vi "GDSLvIcon_AnalyseViIcon.vi"(1 "ViRef/LvCLassRef/LvLibRef/ViPath/2D_Image":variant, 3 "DoATextOCR(False)":bool, 5 "error in (no error)":errorcluster) -> (6 "BodyTextColor":u32(colorbox), 7 "Splitter0px":bool, 8 "HeaderTextColor":u32(colorbox), 9 "BodyText(OCR)":string, 10 "FrameColor":u32(colorbox), 11 "HeadText(OCR)":string, 12 "FrameThickness(1)":u32=1, 13 "ValidHeaderIcon":bool, 14 "DefaultIcon":bool, 15 "HeaderIcon":u8[][](array[numeric]) format="%x", 16 "HeaderBkColor":u32(colorbox), 17 "BodyIcon":u8[][](array[numeric]) format="%x", 18 "BodyBkColor":u32(colorbox), 19 "error out":errorcluster)   [LabVIEW 2020]
uses:
  <vilib>/picture/picture.llb/imagedata.ctl
  <vilib>/Utility/miscctls.llb/LVMapReplaceAction.ctl
  <vilib>/Analysis/NI_AALBase.lvlib
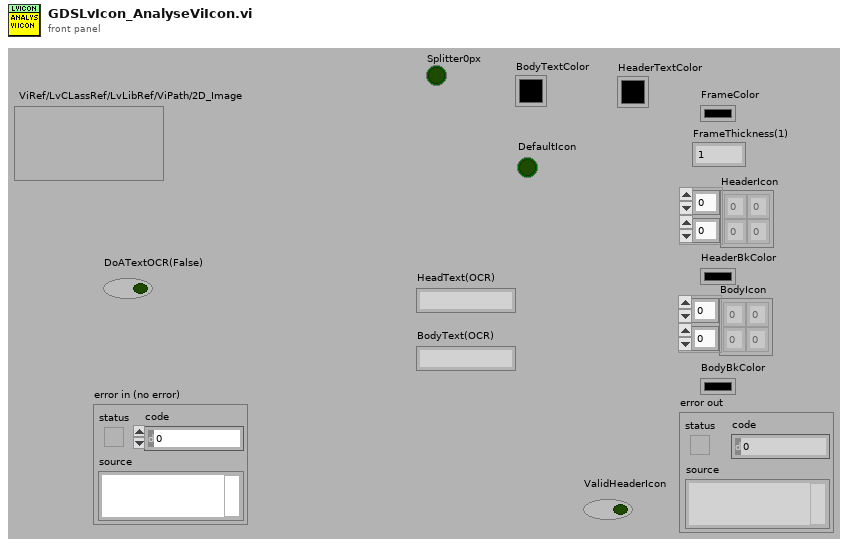
[diagram p1: front panel]
types:
  T1 = cluster{"image":u8[][], "FrameThickness":i32, "FrameColor":u32, "HeaderBkColor":u32, "BodyBkColor":u32, "SplitterAtRow":i32, "Header":u8[][], "Body":u8[][], "HeadTextColor":u32, "BodyTextColor":u32, "BodyBack(8bit)":u8, "BodyText(OCR)":string, "HeadText(OCR)":string, "HeaderBack(8bit)":u8, "EndRow":i32, "StartRow":i32, "BodyTextColor(8bit)":u8, "HeaderTextColor(8bit)":u8, "ShouldHaveHeader":bool, "Splitter0px":bool}
  T2 = typedef "imagedata.ctl" = cluster{"image type":i32, "image depth":i32, "image":u8[], "mask":u8[], "colors":u32[], "Rectangle":cluster{"left":i16, "top":i16, "right":i16, "bottom":i16}}
  T3 = typedef "LVMapReplaceAction.ctl" = enum32{"Modify Entry only if found", "Add or Modify Entry", "Delete Entry"}
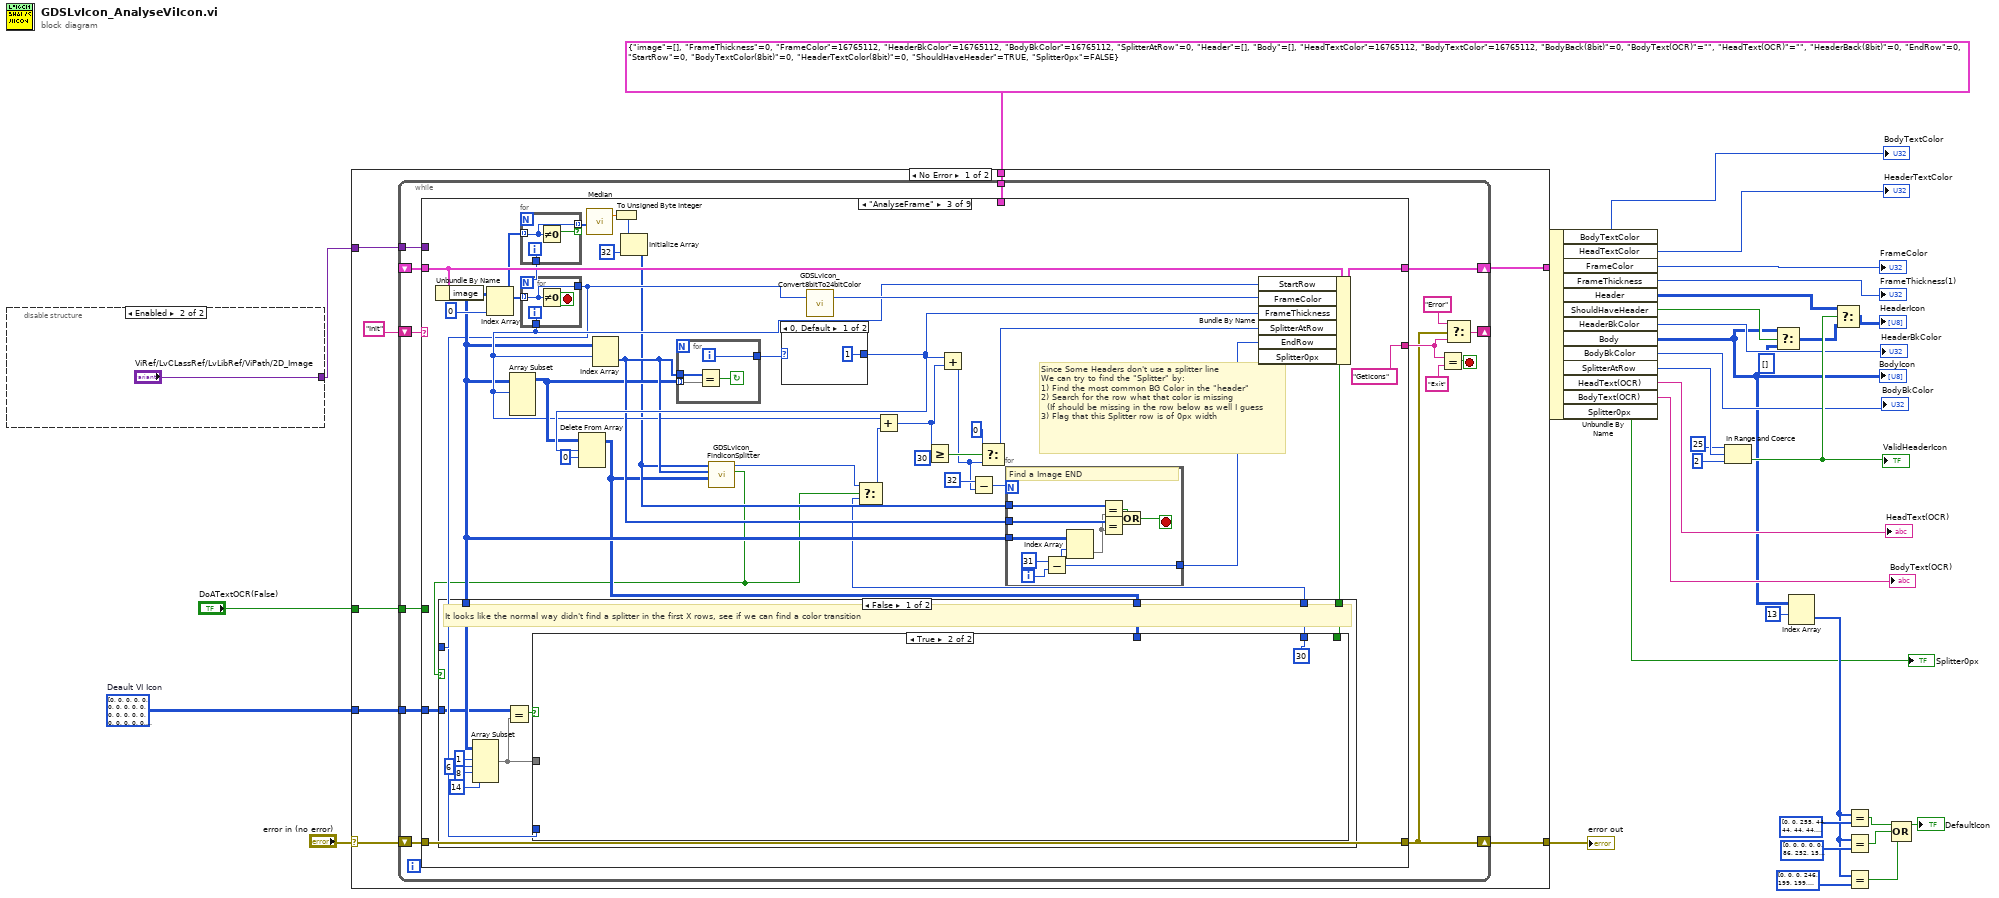
[diagram p0: block diagram]
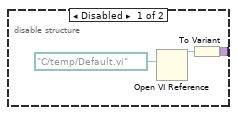
[diagram p2: hidden frame]
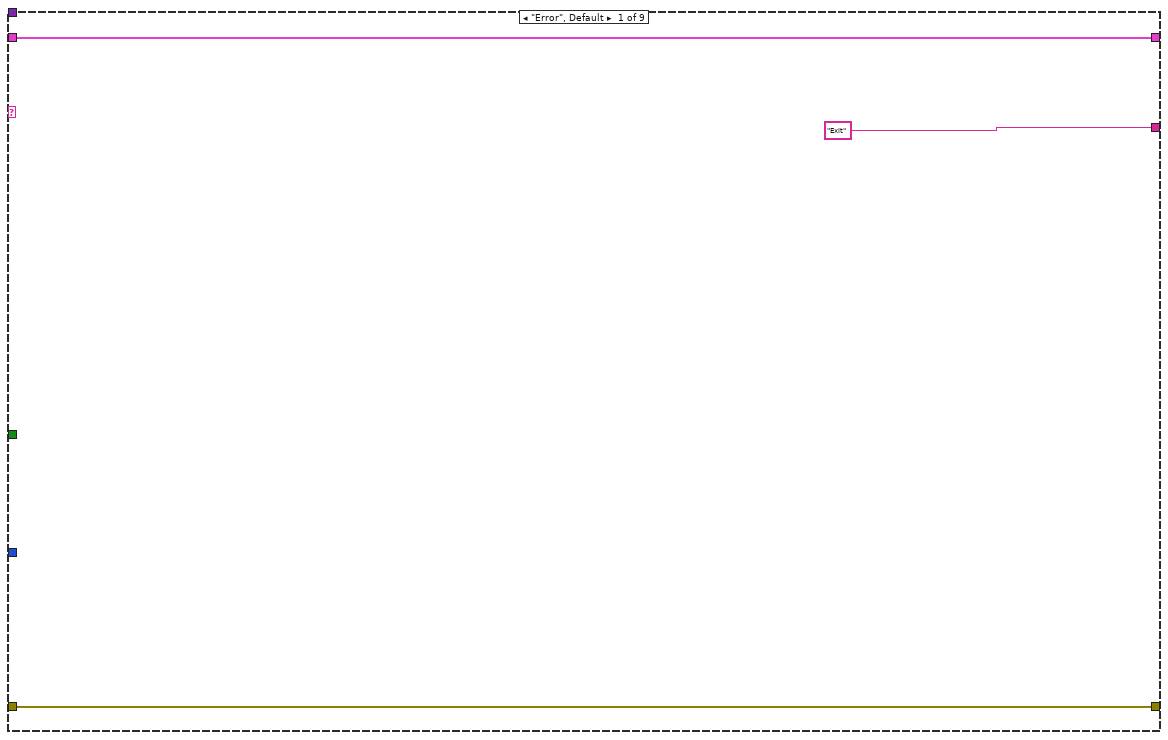
[diagram p3: hidden frame]
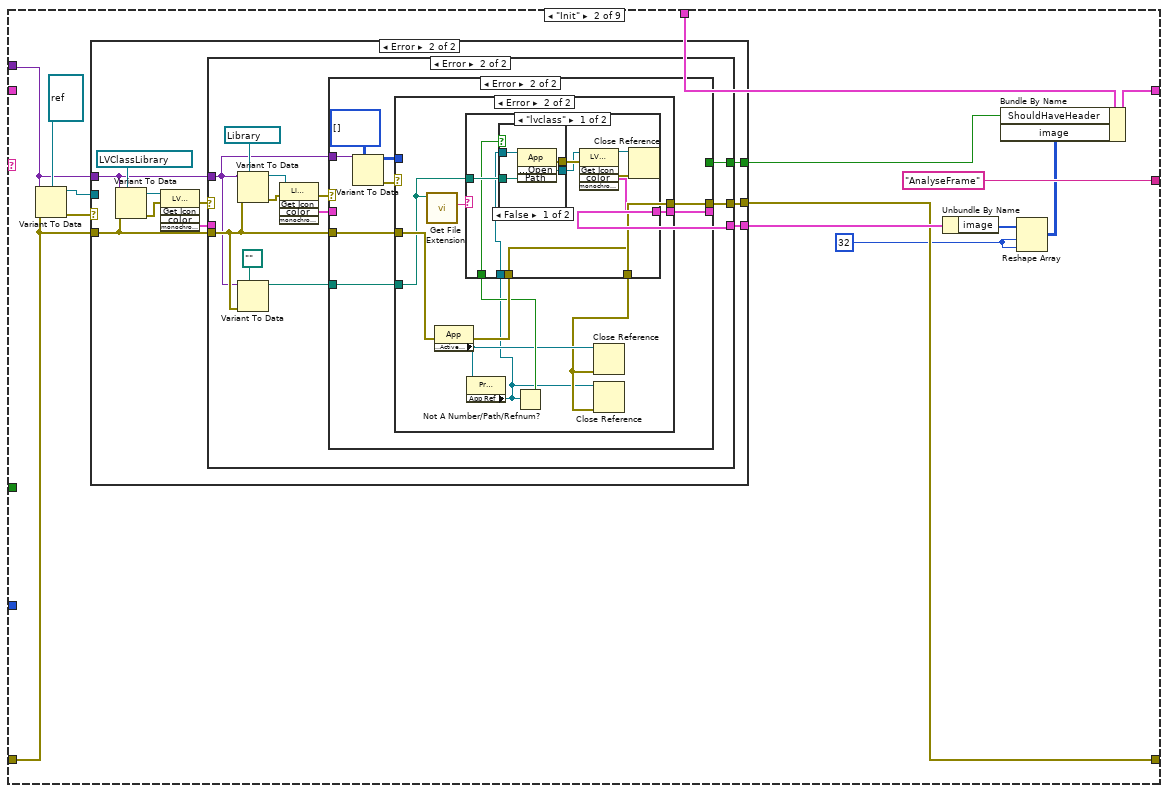
[diagram p4: hidden frame]
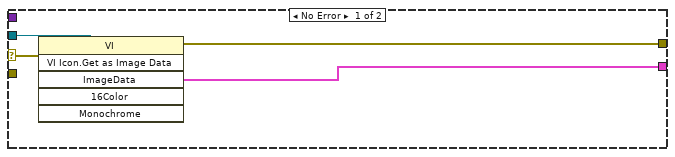
[diagram p5: hidden frame]
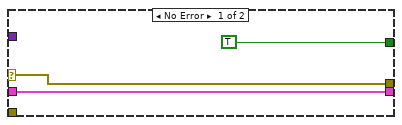
[diagram p7: hidden frame]
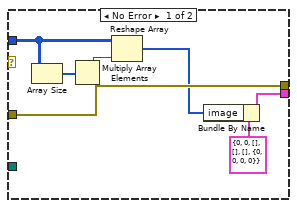
[diagram p8: hidden frame]
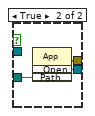
[diagram p9: hidden frame]
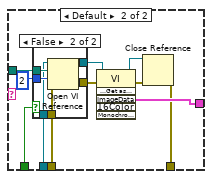
[diagram p10: hidden frame]
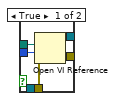
[diagram p11: hidden frame]
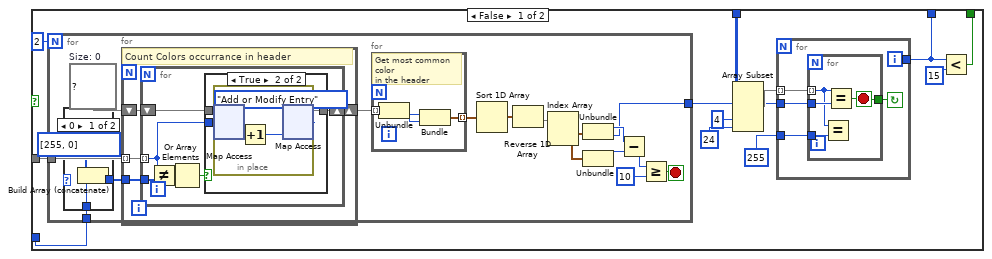
[diagram p12: hidden frame]
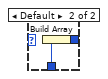
[diagram p13: hidden frame]
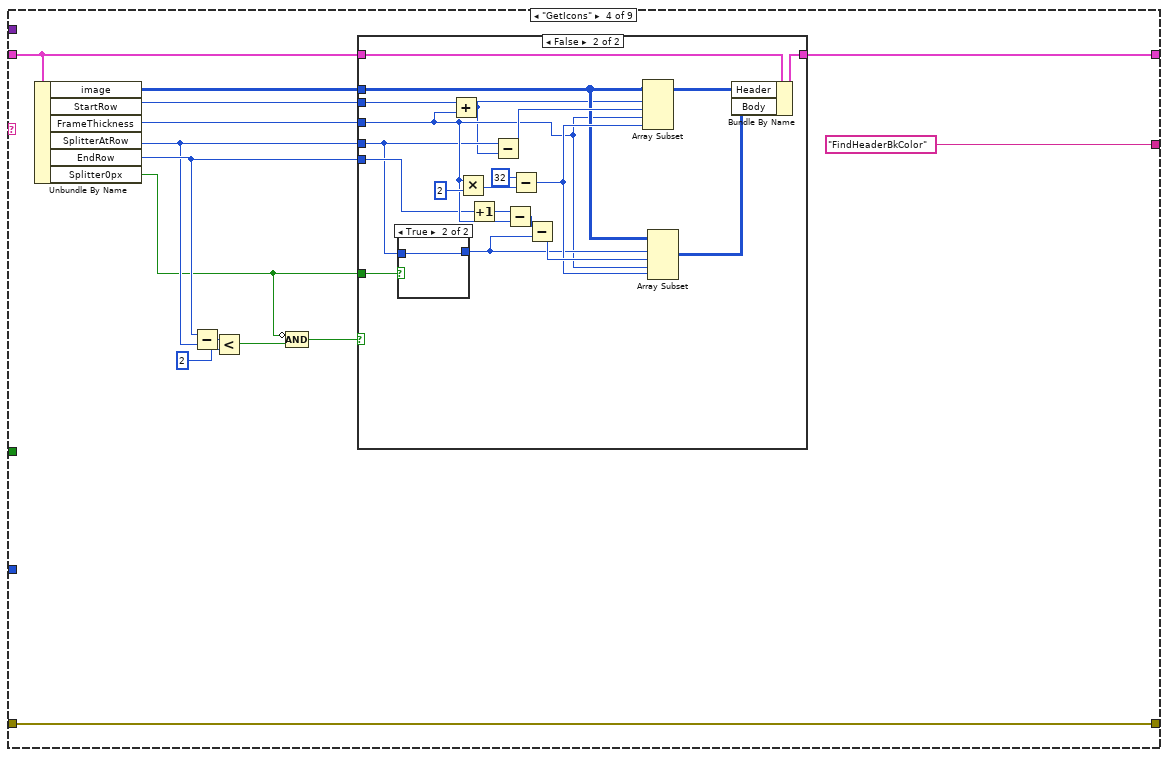
[diagram p17: hidden frame]
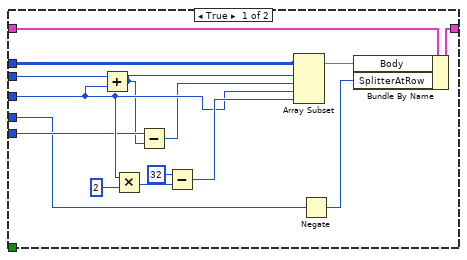
[diagram p18: hidden frame]
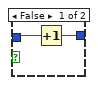
[diagram p19: hidden frame]
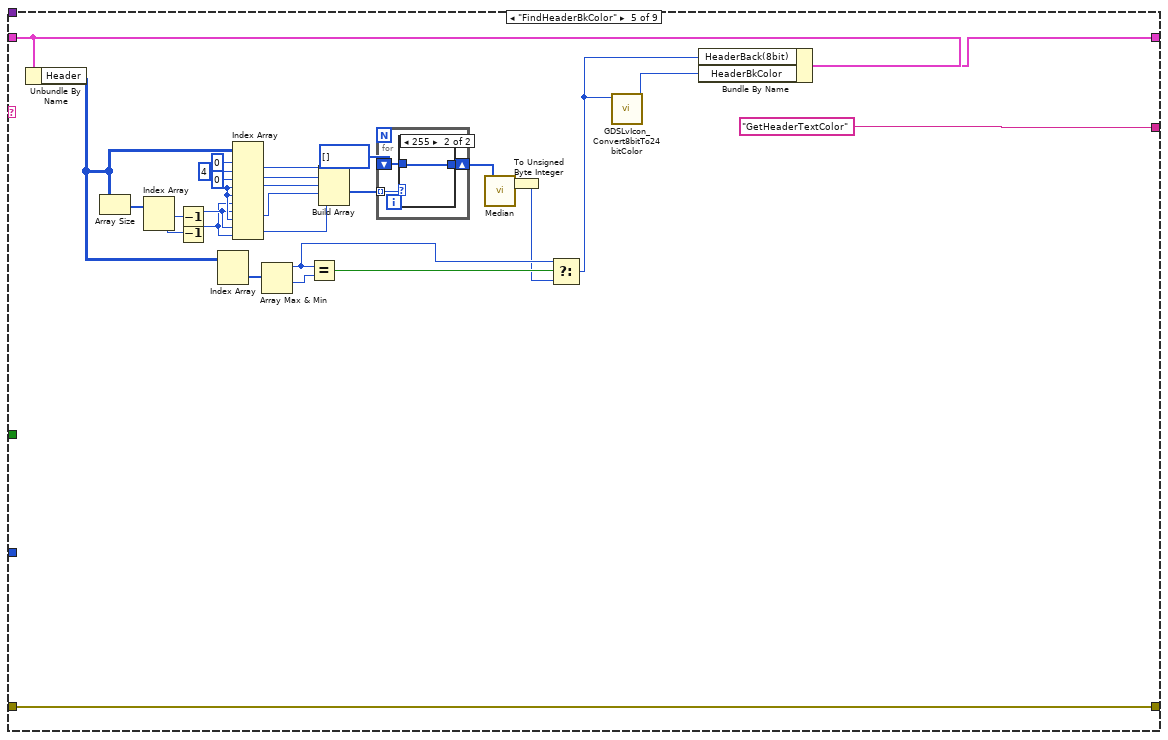
[diagram p20: hidden frame]
diagram:
  w1 = u8[][] [[0, 0, 0, 0, 0, 0, 0, 0, 0, 0, 0, 0, 0, 0], [0, 0, 0, 0, 0, 0, 0, 0, 0, 0, 0, 0, 0, 0], [255, 255, 255, 255, 255, 255, 255, 255, 255, 255, 255, 255, 255, 255], [249, 249, 249, 249, 249, 249, 249, 249, 247, 249, 44, 249, 44, 224], [255, 255, 255, 255, 255, 255, 255, 255, 247, 249, 44, 249, 44, 255], [232, 255, 255, 255, 232, 228, 232, 255, 247, 252, 43, 252, 44, 255]]  # Deault VI Icon
  n1 = disable-structure shown="Enabled" {
    disable-tunnel: [w36 "ViRef/LvCLassRef/LvLibRef/ViPath/2D_Image"] -> w16
    frame Disabled {
      n2 = Open VI Reference(vi path=path "C:/temp/Default.vi") -> (vi reference=w38:refnum<vi>)  [unwired: 5 in, 1 out]
      n3 = To Variant(anything=w38) -> (Variant=w36:variant)
    }
    frame Enabled {
    }
  }
  n4 = case shown="No Error" "error in (no error)" {
    selector: "error in (no error)" -> [w46 w528]
    tunnel: w16 -> [w44 _]
    tunnel: [w45 w528] -> w34
    tunnel: [w43 _] -> w33
    tunnel: T1 {"image"=[], "FrameThickness"=0, "FrameColor"=16765112, "HeaderBkColor"=16765112, "BodyBkColor"=16765112, "SplitterAtRow"=0, "Header"=[], "Body"=[], "HeadTextColor"=16765112, "BodyTextColor"=16765112, "BodyBack(8bit)"=0, "BodyText(OCR)"="", "HeadText(OCR)"="", "HeaderBack(8bit)"=0, "EndRow"=0, "StartRow"=0, "BodyTextColor(8bit)"=0, "HeaderTextColor(8bit)"=0, "ShouldHaveHeader"=TRUE, "Splitter0px"=FALSE} -> [w42 _]
    tunnel: "DoATextOCR(False)" -> [w41 _]
    tunnel: w1 -> [w40 _]
    frame No Error {
      n5 = while {
        shift-right: [w54] -> w45
        shift-left: w46 -> [w61]
        shift-right: [w59] -> _
        shift-left: "Init" -> [w60]
        shift-right: [w53] -> w43
        shift-left: _ -> [w52]
        tunnel: w44 -> [w51]
        tunnel: w42 -> [w50]
        tunnel: w41 -> [w49]
        tunnel: w40 -> [w48]
        stop <- w58 stop-if-true
        n6 = case shown="\"AnalyseFrame\"" w60 {
          tunnel: w61 -> [w64 w68 w204 w318 w387 w409 w442 w471 w512]
          tunnel: [w64 w67 w204 w318 w387 w409 w442 w471 w512] -> w54
          tunnel: ["Exit" "AnalyseFrame" "GetIcons" "FindHeaderBkColor" "GetHeaderTextColor" "FindBodyBkColor" "GetBodyTextColor" w462 "Exit"] -> w55
          tunnel: [w62 w76 w207 w320 w385 w407 w440 w469 w517] -> w53
          tunnel: w52 -> [w62 _ w208 w321 w386 w408 w441 w470 w515]
          tunnel: w51 -> [_ w71 _ _ _ _ _ _ _]
          tunnel: w50 -> [_ w74 _ _ _ _ _ _ _]
          tunnel: w49 -> [_ _ _ _ _ _ _ w464 _]
          tunnel: w48 -> [_ _ w172 _ _ _ _ _ _]
          frame "Error", Default {
          }
          frame "Init" {
            w65 = 32 ("dimension size")
            n7 = Variant To Data(error in=w68, type=refnum<vi> refnum ("ViRef or LvCLassRef"), Variant=w71) -> (data=w70:refnum<vi>, error out=w72:errorcluster)
            n8 = case shown="Error" w72 {
              selector: w72 -> [w81 _]
              tunnel: w71 -> [_ w85]
              tunnel: w70 -> [w82 _]
              tunnel: [w80 w86] -> w69
              tunnel: w68 -> [_ w84]
              tunnel: [w79 w88] -> w67
              tunnel: [_ w83] -> w66
              frame No Error {
                n9 = invoke class="VI" method="VI Icon.Get as Image Data"(reference=w82, error in=w81) -> (error out=w79:errorcluster, "ImageData"=w80:T2)  [unwired: 4 in, 4 out]
              }
              frame Error {
                n10 = Variant To Data(error in=w84, type=refnum<vi> refnum ("LVClassLibrary Refnum"), Variant=w85) -> (data=w91:refnum<vi>, error out=w90:errorcluster)
                n11 = invoke class="LVClassLibrary" method="Get Icon"(reference=w91, error in=w90) -> (error out=w89:errorcluster, "color"=w87:T2)  [unwired: 3 in, 3 out]
                n12 = case shown="Error" w89 {
                  selector: w89 -> [w94 _]
                  tunnel: [w94 w100] -> w88
                  tunnel: w87 -> [w93 _]
                  tunnel: [w93 w101] -> w86
                  tunnel: w85 -> [_ w95]
                  tunnel: w84 -> [_ w97]
                  tunnel: [_ w96] -> w83
                  frame No Error {
                  }
                  frame Error {
                    n13 = Variant To Data(error in=w97, type=refnum<vi> refnum ("Library Refnum"), Variant=w95) -> (data=w105:refnum<vi>, error out=w104:errorcluster)
                    n14 = Variant To Data(error in=w97, type=path "", Variant=w95) -> (data=w98:path)  [unwired: 1 out]
                    n15 = invoke class="Library" method="Get Icon"(reference=w105, error in=w104) -> (error out=w103:errorcluster, "color"=w102:T2)  [unwired: 3 in, 3 out]
                    n16 = case shown="Error" w103 {
                      selector: w103 -> [w108 _]
                      tunnel: w102 -> [w109 _]
                      tunnel: [w109 w116] -> w101
                      tunnel: [w108 w114] -> w100
                      tunnel: w98 -> [_ w117]
                      tunnel: w97 -> [_ w115]
                      tunnel: [TRUE _] -> w96
                      tunnel: w95 -> [_ w113]
                      frame No Error {
                      }
                      frame Error {
                        n17 = Variant To Data(type=u8[][] [] ("output array"), Variant=w113) -> (data=w110:u8[][], error out=w111:errorcluster)  [unwired: 1 in]
                        n18 = case shown="Error" w111 {
                          tunnel: w117 -> [_ w126]
                          tunnel: [w122 w133] -> w116
                          tunnel: w115 -> [w124 w127]
                          tunnel: [w124 w129] -> w114
                          tunnel: w110 -> [w121 _]
                          frame No Error {
                            n19 = Array Size(array=w121) -> (size(s)=w119:i32[])
                            n20 = Multiply Array Elements(1:w119) -> (0:w120:i32)
                            n21 = Reshape Array(w121, w120) -> (w118:u8[])
                            n22 = Bundle By Name(cluster=T2 {"image type"=0, "image depth"=0, "image"=[], "mask"=[], "colors"=[], "Rectangle"={"left"=0, "top"=0, "right"=0, "bottom"=0}} ("ImageData"), "image"=w118) -> (w122:T2)
                          }
                          frame Error {
                            n23 = call <vilib>:"Get File Extension.vi"("file"=w126) -> ("lowercase file extension"=w125:string)  [unwired: 6 in, 4 out]
                            n24 = property class="App"(error in=w127) -> (error out=w132:errorcluster, "Project:Active Project"=w130:refnum<vi>)  [unwired: 1 in, 1 out]
                            n25 = property class="Project"(reference=w130) -> ("App Ref"=w128:refnum<vi>)  [unwired: 1 in, 2 out]
                            n26 = Not A Number/Path/Refnum?(number/path/refnum=w128) -> (NaN/Path/Refnum?=w131:bool)
                            n27 = case shown="\"lvclass\"" w125 {
                              tunnel: [w138 w156] -> w133
                              tunnel: w132 -> [w134 w154]
                              tunnel: w131 -> [w135 w153]
                              tunnel: [w134 w152] -> w129
                              tunnel: w128 -> [w139 w151]
                              tunnel: w126 -> [w140 w150]
                              frame "lvclass" {
                                n28 = case shown="False" w135 {
                                tunnel: [w146 w149] -> w142
                                tunnel: [w145 w148] -> w141
                                tunnel: w140 -> [w144 w147]
                                tunnel: w139 -> [w143 _]
                                frame False {
                                n29 = invoke class="App" method="LVClass.Open"(reference=w143, "Path"=w144) -> (error out=w146:errorcluster, "LVClass.Open"=w145:refnum<vi>)  [unwired: 2 in, 2 out]
                                }
                                frame True {
                                n30 = invoke class="App" method="LVClass.Open"("Path"=w147) -> (error out=w149:errorcluster, "LVClass.Open"=w148:refnum<vi>)  [unwired: 3 in, 2 out]
                                }
                                }
                                n31 = invoke class="LVClassLibrary" method="Get Icon"(reference=w141, error in=w142) -> (reference out=w136:refnum<vi>, error out=w137:errorcluster, "color"=w138:T2)  [unwired: 3 in, 2 out]
                                n32 = Close Reference(reference=w136, error in (no error)=w137) -> ()  [unwired: 1 out]
                              }
                              frame Default {
                                n33 = case shown="False" w153 {
                                tunnel: w150 -> [w165 w171]
                                tunnel: [w164 w170] -> w160
                                tunnel: [w163 w169] -> w159
                                tunnel: 2 ("options") -> [w162 w168]
                                tunnel: w154 -> [w161 w167]
                                tunnel: w151 -> [_ w166]
                                frame True {
                                n34 = Open VI Reference(vi path=w165, options=w162, error in (no error)=w161) -> (vi reference=w163:refnum<vi>, error out=w164:errorcluster)  [unwired: 3 in]
                                }
                                frame False {
                                n35 = Open VI Reference(application reference (local)=w166, vi path=w171, options=w168, error in (no error)=w167) -> (vi reference=w169:refnum<vi>, error out=w170:errorcluster)  [unwired: 2 in]
                                }
                                }
                                n36 = invoke class="VI" method="VI Icon.Get as Image Data"(reference=w159, error in=w160) -> (reference out=w157:refnum<vi>, error out=w158:errorcluster, "ImageData"=w156:T2)  [unwired: 4 in, 3 out]
                                n37 = Close Reference(reference=w157, error in (no error)=w158) -> (error out=w152:errorcluster)
                              }
                            }
                            n38 = Close Reference(reference=w130, error in (no error)=w129) -> ()  [unwired: 1 out]
                            n39 = Close Reference(reference=w128, error in (no error)=w129) -> ()  [unwired: 1 out]
                          }
                        }
                      }
                    }
                  }
                }
              }
            }
            n40 = Unbundle By Name(w69) -> ("image"=w77:u8[])
            n41 = Reshape Array(w77, w65, w65) -> (w75:u8[][])
            n42 = Bundle By Name(cluster=w74, "ShouldHaveHeader"=w66, "image"=w75) -> (w76:T1)
          }
          frame "AnalyseFrame" {
            # "Since Some Headers don't use a splitter line\nWe can try to find the \"Splitter\" by:\n1) Find the most common BG Color in the \"header\"\n2) Search for the row what that color is missing\n  (If should be missing in the row below as well I guess\n3) Flag that this Splitter row is of 0px width"
            n43 = Unbundle By Name(w208) -> ("image"=w188:u8[][])
            n44 = Index Array(array=w188, index (col)=0 ("index (row)")) -> (element=w185:u8[])  [unwired: 1 in]
            n45 = for {
              tunnel: w185 -> [w288] mode=indexing
              tunnel: [w288] -> w184 mode=indexing if=w286
              tunnel: [w287] -> w186
              i -> [w287]
              n46 = Not Equal To 0?(x=w288) -> (x != 0?=w286:bool)
            }
            n47 = for {
              N: w186 -> [_]
              tunnel: w185 -> [w290] mode=indexing
              tunnel: [w290] -> w187
              tunnel: [w289] -> w190
              i -> [w289]
              stop <- w291 stop-if-true
              n48 = Not Equal To 0?(x=w290) -> (x != 0?=w291:bool)
            }
            n49 = Array Subset(array=w188, index (row)=w190) -> (w192:u8[][])  [unwired: 3 in]
            n50 = call <vilib>:"Median.vi"("X"=w184) -> ("median"=w182:dbl)  [unwired: 1 out]
            n51 = Index Array(array=w188, index (row)=w190) -> (element=w196:u8[])  [unwired: 1 in]
            n52 = To Unsigned Byte Integer(number=w182) -> (unsigned 8bit integer=w181:u8)
            n53 = Initialize Array(w181, 32 ("dimension size")) -> (w180:u8[])
            n54 = for {
              tunnel: w192 -> [w305] mode=indexing
              tunnel: w196 -> [w304]
              tunnel: [w303] -> w203
              i -> [w303]
              stop <- w302 continue-if-true
              n55 = Equal?(x=w304, y=w305) -> (x = y?=w302:bool)
            }
            n56 = case shown="0, Default" w203 {
              selector: w203 -> [_ w307]
              tunnel: [1 w307] -> w202
              frame 0, Default {
              }
              frame 1..3 {
              }
            }
            n57 = Delete From Array(array=w192, length=w202, index (row)=0) -> (array with subset deleted=w179:u8[][])  [unwired: 1 in, 1 out]
            n58 = call <resource>:"GDSLvIcon_FindIconSplitter.vi"("Icon(Top Frame Rows removed)"=w179, "SolidTopRow'sMost Common Color)"=w196, "TopRow(Frame)"=w180) -> ("Splitter probably found"=w178:bool, "Splitter Index found (-(FrameThickness), since the Icon in is missing the Frame)"=w176:i32)  [unwired: 7 in]
            n59 = case shown="False" w178 {
              tunnel: w188 -> [w220 _]
              tunnel: w187 -> [w215 _]
              tunnel: w179 -> [w214 _]
              tunnel: [w213 _] -> w177
              tunnel: [w212 _] -> w174
              tunnel: w172 -> [w210 _]
              frame False {
                # "It looks like the normal way didn't find a splitter in the first X rows, see if we can find a color transition"
                n60 = Array Subset(array=w220, index (row)=1 ("index"), length (row)=6 ("length"), index (col)=8 ("index"), length (col)=14 ("length")) -> (w211:u8[][])
                n61 = Equal?(x=w210, y=w211) -> (x = y?=w209:bool)
                n62 = case shown="True" w209 {
                  tunnel: w215 -> [w232 _]
                  tunnel: w214 -> [w230 _]
                  tunnel: [w225 30] -> w213
                  tunnel: [w224 _] -> w212
                  tunnel: w211 -> [w221 _]
                  frame False {
                    n63 = for {
                      N: 2 -> [_]
                      tunnel: w221 -> [w249]
                      tunnel: w232 -> [w246]
                      tunnel: [w235] -> w223
                      i -> [w233]
                      stop <- w236 stop-if-true
                      w248 = map{u8, i32} {}  # Size: 0
                      n64 = case shown="0" w233 {
                        tunnel: w246 -> [w252 w254]
                        tunnel: [w251 w253] -> w234
                        frame 0 {
                          n65 = Build Array (concatenate)(u8[] [255, 0], w252) -> (w251:u8[])
                        }
                        frame Default {
                          n66 = Build Array(w254) -> (w253:u8[])
                        }
                      }
                      n67 = for {
                        tunnel: w249 -> [w262] mode=indexing
                        shift-right: [w260] -> w247
                        shift-left: w248 -> [w261]
                        tunnel: w234 -> [w259]
                        # "Count Colors occurrance in header"
                        n68 = for {
                          tunnel: w262 -> [w266] mode=indexing
                          shift-right: [w267] -> w260
                          shift-left: w261 -> [w268]
                          tunnel: w259 -> [w265]
                          n69 = Not Equal?(x=w266, y=w265) -> (x != y?=w264:bool[])
                          n70 = Or Array Elements(Boolean array=w264) -> (logical OR=w263:bool)
                          n71 = case shown="True" w263 {
                            tunnel: w268 -> [w269 w272]
                            tunnel: [w269 w271] -> w267
                            tunnel: w266 -> [_ w270]
                            frame False {
                            }
                            frame True {
                              n72 = in-place {
                                n73 = in-place-map #1(w272, w270) -> (w274:i32)  [unwired: 1 in, 1 out]
                                n74 = Increment(x=w274) -> (x+1=w273:i32)
                                n75 = in-place-map #1(w273, LVMapReplaceAction."Add or Modify Entry" ("action")) -> (w271:map{u8, i32})  [unwired: 2 out]
                              }
                            }
                          }
                        }
                      }
                      n76 = for {
                        tunnel: w247 -> [w258] mode=indexing
                        tunnel: [w255] -> w245 mode=indexing
                        # "Get most common color\nin the header"
                        n77 = Unbundle(w258) -> ("Colour"=w256:u8, "Counts"=w257:i32)
                        n78 = Bundle("Counts"=w257, "Colour"=w256) -> (w255:cluster{"Counts":i32, "Colour":u8})  [unwired: 1 in]
                      }
                      n79 = Sort 1D Array(array=w245) -> (sorted array=w244:cluster{"Counts":i32, "Colour":u8}[])
                      n80 = Reverse 1D Array(array=w244) -> (reversed array=w243:cluster{"Counts":i32, "Colour":u8}[])
                      n81 = Index Array(array=w243) -> (element #1=w242:cluster{"Counts":i32, "Colour":u8}, element #2=w241:cluster{"Counts":i32, "Colour":u8})  [unwired: 2 in]
                      n82 = Unbundle(w242) -> ("Counts"=w240:i32, "Colour"=w235:u8)
                      n83 = Unbundle(w241) -> ("Counts"=w239:i32)  [unwired: 1 out]
                      n84 = Subtract(x=w240, y=w239) -> (x-y=w238:i32)
                      n85 = Greater Or Equal?(x=w238, y=10) -> (x >= y?=w236:bool)
                    }
                    n86 = Array Subset(array=w230, index (col)=4 ("index"), length (col)=24 ("length")) -> (w227:u8[][])  [unwired: 2 in]
                    n87 = for {
                      tunnel: w227 -> [w280] mode=indexing
                      tunnel: w223 -> [w279]
                      tunnel: u8 255 -> [w278]
                      tunnel: [w276] -> w225
                      i -> [w276]
                      stop <- w277 continue-if-true
                      n88 = for {
                        tunnel: w280 -> [w283] mode=indexing
                        tunnel: w279 -> [w284]
                        tunnel: w278 -> [w282]
                        tunnel: [w281] -> w277
                        stop <- w281 stop-if-true
                        n89 = Equal?(x=w283, y=w282) -> ()  [unwired: 1 out]
                        n90 = Equal?(x=w283, y=w284) -> (x = y?=w281:bool)
                      }
                    }
                    n91 = Less?(x=w225, y=15) -> (x < y?=w224:bool)
                  }
                  frame True {
                  }
                }
              }
              frame True {
              }
            }
            n92 = call <resource>:"GDSLvIcon_Convert8bitTo24bitColor.vi"("Color8bit"=w187) -> ("Color24bit"=w197:u32)  [unwired: 17 in, 1 out]
            n93 = Select(t=w176, s=w178, f=w177) -> (s? t:f=w175:i32)
            n94 = Add(x=w190, y=w175) -> (x+y=w189:i32)
            n95 = Greater Or Equal?(x=w189, y=30) -> (x >= y?=w200:bool)
            n96 = Add(x=w202, y=w189) -> (x+y=w173:i32)
            n97 = Subtract(x=32 ("y"), y=w173) -> (x-y=w194:i32)
            n98 = Select(t=0, s=w200, f=w173) -> (s? t:f=w198:i32)
            n99 = for {
              N: w194 -> [_]
              tunnel: w196 -> [w301]
              tunnel: w188 -> [w298]
              tunnel: [w297] -> w191
              tunnel: w180 -> [w295]
              i -> [w299]
              stop <- w292 stop-if-true
              # "Find a Image END"
              n100 = Subtract(x=31 ("y"), y=w299) -> (x-y=w297:i32)
              n101 = Index Array(array=w298, index (row)=w297) -> (element=w296:u8[])  [unwired: 1 in]
              n102 = Equal?(x=w295, y=w296) -> (x = y?=w294:bool)
              n103 = Equal?(x=w301, y=w296) -> (x = y?=w293:bool)
              n104 = Or(x=w294, y=w293) -> (x .or. y?=w292:bool)
            }
            n105 = Bundle By Name(cluster=w208, "StartRow"=w190, "FrameColor"=w197, "FrameThickness"=w202, "SplitterAtRow"=w198, "EndRow"=w191, "Splitter0px"=w174) -> (w207:T1)
          }
          frame "GetIcons" {
            n106 = Unbundle By Name(w321) -> ("image"=w317:u8[][], "StartRow"=w315:i32, "FrameThickness"=w316:i32, "SplitterAtRow"=w313:i32, "EndRow"=w314:i32, "Splitter0px"=w308:bool)
            n107 = Subtract(x=w314, y=w313) -> (x-y=w312:i32)
            n108 = Less?(x=w312, y=2) -> (x < y?=w311:bool)
            n109 = Compound Arithmetic op=AND(invert w308, w311) -> (w309:bool)
            n110 = case shown="False" w309 {
              tunnel: w321 -> [w336 w356]
              tunnel: [w335 w355] -> w320
              tunnel: w317 -> [w329 w344]
              tunnel: w316 -> [w328 w343]
              tunnel: w315 -> [w327 w342]
              tunnel: w314 -> [w326 w341]
              tunnel: w313 -> [w323 w340]
              tunnel: w308 -> [_ w337]
              frame True {
                n111 = Add(x=w327, y=w328) -> (x+y=w325:i32)
                n112 = Multiply(x=w328, y=2) -> (x*y=w332:i32)
                n113 = Subtract(x=w326, y=w325) -> (x-y=w324:i32)
                n114 = Subtract(x=32, y=w332) -> (x-y=w331:i32)
                n115 = Array Subset(array=w329, index (row)=w325, length (row)=w324, index (col)=w328, length (col)=w331) -> (w334:u8[][])
                n116 = Negate(x=w323) -> (-x=w322:i32)
                n117 = Bundle By Name(cluster=w336, "Body"=w334, "SplitterAtRow"=w322) -> (w335:T1)
              }
              frame False {
                n118 = case shown="True" w337 {
                  tunnel: [w358 w359] -> w345
                  tunnel: w340 -> [w357 w359]
                  frame False {
                    n119 = Increment(x=w357) -> (x+1=w358:i32)
                  }
                  frame True {
                  }
                }
                n120 = Add(x=w342, y=w343) -> (x+y=w339:i32)
                n121 = Multiply(x=w343, y=2) -> (x*y=w351:i32)
                n122 = Increment(x=w341) -> (x+1=w338:i32)
                n123 = Subtract(x=w340, y=w339) -> (x-y=w353:i32)
                n124 = Subtract(x=w338, y=w343) -> (x-y=w346:i32)
                n125 = Subtract(x=32, y=w351) -> (x-y=w349:i32)
                n126 = Subtract(x=w346, y=w345) -> (x-y=w350:i32)
                n127 = Array Subset(array=w344, index (row)=w339, length (row)=w353, index (col)=w343, length (col)=w349) -> (w354:u8[][])
                n128 = Array Subset(array=w344, index (row)=w345, length (row)=w350, index (col)=w343, length (col)=w349) -> (w348:u8[][])
                n129 = Bundle By Name(cluster=w356, "Header"=w354, "Body"=w348) -> (w355:T1)
              }
            }
          }
          frame "FindHeaderBkColor" {
            w380 = 0 ("index (row)")
            n130 = Unbundle By Name(w386) -> ("Header"=w362:u8[][])
            n131 = Array Size(array=w362) -> (size(s)=w383:i32[])
            n132 = Index Array(array=w383) -> (element #1=w382:i32, element #2=w381:i32)  [unwired: 2 in]
            n133 = Decrement(x=w382) -> (x-1=w379:i32)
            n134 = Decrement(x=w381) -> (x-1=w378:i32)
            n135 = Index Array(array=w362) -> (element=w373:u8[])  [unwired: 2 in]
            n136 = Index Array(array=w362, index (row) #1=0 ("index (row)"), index (col) #1=4 ("disabled index (col)"), index (row) #2=w380, index (col) #2=w380, index (row) #3=w380, index (col) #3=w378, index (row) #4=w379, index (col) #4=w380, index (row) #5=w379, index (col) #5=w378) -> (element #1=w366:u8, element #2=w377:u8, element #3=w376:u8, element #4=w375:u8, element #5=w374:u8)
            n137 = Array Max & Min(array=w373) -> (max value=w370:u8, min value=w372:u8)  [unwired: 2 out]
            n138 = Equal?(x=w370, y=w372) -> (x = y?=w371:bool)
            n139 = Build Array(w366, w377, w376, w375, w374) -> (w365:u8[])
            n140 = for {
              tunnel: w365 -> [w391] mode=indexing
              shift-right: [w389] -> w363
              shift-left: u8[] [] -> [w390]
              n141 = case shown="255" w391 {
                selector: w391 -> [w392 _]
                tunnel: w390 -> [w394 w395]
                tunnel: [w393 w395] -> w389
                frame Default {
                  n142 = Build Array (concatenate)(w394, w392) -> (w393:u8[])
                }
                frame 255 {
                }
              }
            }
            n143 = call <vilib>:"Median.vi"("X"=w363) -> ("median"=w369:dbl)  [unwired: 1 out]
            n144 = To Unsigned Byte Integer(number=w369) -> (unsigned 8bit integer=w360:u8)
            n145 = Select(t=w370, s=w371, f=w360) -> (s? t:f=w361:u8)
            n146 = call <resource>:"GDSLvIcon_Convert8bitTo24bitColor.vi"("Color8bit"=w361) -> ("Color24bit"=w384:u32)  [unwired: 17 in, 1 out]
            n147 = Bundle By Name(cluster=w386, "HeaderBack(8bit)"=w361, "HeaderBkColor"=w384) -> (w385:T1)
          }
          frame "GetHeaderTextColor" {
            w397 = u8 255  # Black(8bit)
            n148 = Unbundle By Name(w408) -> ("HeaderBack(8bit)"=w402:u8, "Header"=w405:u8[][])
            n149 = Array Size(array=w405) -> (size(s)=w404:i32[])
            n150 = Multiply Array Elements(1:w404) -> (0:w401:i32)
            n151 = Reshape Array(w405, w401) -> (w403:u8[])
            n152 = Decrement(x=w401) -> (x-1=w400:i32)
            n153 = for {
              tunnel: w403 -> [w412] mode=indexing
              tunnel: w402 -> [w413]
              tunnel: w400 -> [_]
              tunnel: [w411] -> w399
              tunnel: [w412] -> w398
              stop <- w411 stop-if-true
              n154 = Not Equal?(x=w413, y=w412) -> (x != y?=w411:bool)
            }
            n155 = Select(t=w398, s=w399, f=w397) -> (s? t:f=w396:u8)
            n156 = call <resource>:"GDSLvIcon_Convert8bitTo24bitColor.vi"("Color8bit"=w396) -> ("Color24bit"=w406:u32)  [unwired: 17 in, 1 out]
            n157 = Bundle By Name(cluster=w408, "HeaderTextColor(8bit)"=w396, "HeadTextColor"=w406) -> (w407:T1)
          }
          frame "FindBodyBkColor" {
            w436 = 0 ("index (row)")
            n158 = Unbundle By Name(w441) -> ("Body"=w427:u8[][])  [unwired: 1 out]
            n159 = Array Size(array=w427) -> (size(s)=w439:i32[])
            n160 = Index Array(array=w439) -> (element #1=w438:i32, element #2=w437:i32)  [unwired: 2 in]
            n161 = Decrement(x=w438) -> (x-1=w435:i32)
            n162 = Decrement(x=w437) -> (x-1=w434:i32)
            n163 = Index Array(array=w427) -> (element=w426:u8[])  [unwired: 2 in]
            n164 = Index Array(array=w427, index (row) #1=0 ("index (row)"), index (col) #1=4 ("disabled index (col)"), index (row) #2=w436, index (col) #2=w436, index (row) #3=w436, index (col) #3=w434, index (row) #4=w435, index (col) #4=w436, index (row) #5=w435, index (col) #5=w434) -> (element #1=w418:u8, element #2=w433:u8, element #3=w432:u8, element #4=w431:u8, element #5=w430:u8)
            n165 = Array Max & Min(array=w426) -> (max value=w423:u8, min value=w425:u8)  [unwired: 2 out]
            n166 = Equal?(x=w423, y=w425) -> (x = y?=w424:bool)
            n167 = Build Array(w418, w433, w432, w431, w430) -> (w417:u8[])
            n168 = for {
              tunnel: w417 -> [w445] mode=indexing
              shift-right: [w443] -> w415
              shift-left: u8[] [] -> [w444]
              n169 = case shown="255" w445 {
                selector: w445 -> [w446 _]
                tunnel: w444 -> [w448 w449]
                tunnel: [w447 w449] -> w443
                frame Default {
                  n170 = Build Array (concatenate)(w448, w446) -> (w447:u8[])
                }
                frame 255 {
                }
              }
            }
            n171 = call <vilib>:"Median.vi"("X"=w415) -> ("median"=w422:dbl)  [unwired: 1 out]
            n172 = To Unsigned Byte Integer(number=w422) -> (unsigned 8bit integer=w414:u8)
            n173 = Select(t=w423, s=w424, f=w414) -> (s? t:f=w421:u8)
            n174 = call <resource>:"GDSLvIcon_Convert8bitTo24bitColor.vi"("Color8bit"=w421) -> ("Color24bit"=w429:u32)  [unwired: 17 in, 1 out]
            n175 = Bundle By Name(cluster=w441, "BodyBack(8bit)"=w421, "BodyBkColor"=w429) -> (w440:T1)
          }
          frame "GetBodyTextColor" {
            w460 = u8 255  # Black(8bit)
            n176 = Unbundle By Name(w470) -> ("BodyBack(8bit)"=w467:u8, "Body"=w453:u8[][])
            n177 = for {
              N: 2 -> [_]
              tunnel: w453 -> [w488]
              tunnel: w467 -> [w492]
              tunnel: [w485] -> w466
              tunnel: [w489] -> w465
              i -> [w486]
              stop <- w485 stop-if-true
              n178 = case shown="0, Default" w486 {
                tunnel: w488 -> [w498 w499]
                tunnel: [w497 w499] -> w487
                frame 0, Default {
                  n179 = Array Subset(array=w498, length (row)=10 ("length"), length (col)=10 ("length")) -> (w497:u8[][])  [unwired: 2 in]
                }
                frame 1 {
                }
              }
              n180 = Array Size(array=w487) -> (size(s)=w494:i32[])
              n181 = Multiply Array Elements(1:w494) -> (0:w491:i32)
              n182 = Reshape Array(w487, w491) -> (w493:u8[])
              n183 = Decrement(x=w491) -> (x-1=w490:i32)
              n184 = for {
                tunnel: w493 -> [w501] mode=indexing
                tunnel: w492 -> [w502]
                tunnel: w490 -> [_]
                tunnel: [w500] -> w485
                tunnel: [w501] -> w489
                stop <- w500 stop-if-true
                n185 = Not Equal?(x=w502, y=w501) -> (x != y?=w500:bool)
              }
            }
            n186 = Select(t=w465, s=w466, f=w460) -> (s? t:f=w457:u8)
            n187 = call <resource>:"GOOP_IconOCR.vi"("BackColor(T), TextColor(F)"=FALSE, "BackColor Or TextColor(8bit)"=w457, "Icon"=w453) -> ("String"=w455:string)  [unwired: 8 in]
            n188 = String Length(string=w455) -> (length=w454:i32)
            n189 = case shown="0, Default" w454 {
              tunnel: w453 -> [w476 _]
              tunnel: u8[] [255, 0, 5] -> [w475 _]
              tunnel: [w473 TRUE] -> w451
              tunnel: [w472 _] -> w450
              frame 0, Default {
                n190 = for {
                  tunnel: w476 -> [w481]
                  tunnel: w475 -> [w477] mode=indexing
                  tunnel: [w478] -> w474
                  tunnel: [w477] -> w472
                  stop <- w478 stop-if-true
                  n191 = call <resource>:"GOOP_IconOCR.vi"("BackColor(T), TextColor(F)"=FALSE, "BackColor Or TextColor(8bit)"=w477, "Icon"=w481) -> ("String"=w483:string)  [unwired: 8 in]
                  n192 = String Length(string=w483) -> (length=w480:i32)
                  n193 = Greater Or Equal?(x=w480, y=2) -> (x >= y?=w478:bool)
                }
                n194 = Not(x=w474) -> (.not. x?=w473:bool)
              }
              frame 2.. {
              }
            }
            n195 = Select(t=w457, s=w451, f=w450) -> (s? t:f=w458:u8)
            n196 = call <resource>:"GDSLvIcon_Convert8bitTo24bitColor.vi"("Color8bit"=w458) -> ("Color24bit"=w468:u32)  [unwired: 17 in, 1 out]
            n197 = Bundle By Name(cluster=w470, "BodyTextColor(8bit)"=w458, "BodyTextColor"=w468) -> (w469:T1)
            n198 = Select(t="OCR", s=w464, f="Exit") -> (s? t:f=w462:string)
          }
          frame "OCR" {
            w504 = bool[] [FALSE, TRUE]
            n199 = Unbundle By Name(w515) -> ("Header"=w508:u8[][], "HeaderTextColor(8bit)"=w506:u8, "HeaderBack(8bit)"=w505:u8)  [unwired: 1 out]
            n200 = Unbundle By Name(w515) -> ("Body"=w513:u8[][], "BodyTextColor(8bit)"=w509:u8, "BodyBack(8bit)"=w510:u8)
            n201 = Build Array(w509, w510) -> (w511:u8[])
            n202 = Build Array(w506, w505) -> (w507:u8[])
            n203 = for {
              tunnel: [w525] -> w514
              tunnel: w513 -> [w527]
              tunnel: w504 -> [w526] mode=indexing
              tunnel: w511 -> [w523] mode=indexing
              stop <- w524 continue-if-true
              n204 = call <resource>:"GOOP_IconOCR.vi"("BackColor(T), TextColor(F)"=w526, "BackColor Or TextColor(8bit)"=w523, "Icon"=w527) -> ("String"=w525:string)  [unwired: 8 in]
              n205 = Empty String/Path?(string/path=w525) -> (empty?=w524:bool)
            }
            n206 = for {
              tunnel: [w520] -> w503
              tunnel: w508 -> [w522]
              tunnel: w504 -> [w521] mode=indexing
              tunnel: w507 -> [w518] mode=indexing
              stop <- w519 continue-if-true
              n207 = call <resource>:"GOOP_IconOCR.vi"("BackColor(T), TextColor(F)"=w521, "BackColor Or TextColor(8bit)"=w518, "Icon"=w522) -> ("String"=w520:string)  [unwired: 8 in]
              n208 = Empty String/Path?(string/path=w520) -> (empty?=w519:bool)
            }
            n209 = Bundle By Name(cluster=w515, "BodyText(OCR)"=w514, "HeadText(OCR)"=w503) -> (w517:T1)
          }
        }
        n210 = Equal?(x=w55, y="Exit") -> (x = y?=w58:bool)
        n211 = Select(t="Error", s=w54, f=w55) -> (s? t:f=w59:string)
      }
    }
    frame Error {
    }
  }
  "error out" <- w34
  n212 = Unbundle By Name(w33) -> ("BodyTextColor"=→"BodyTextColor":u32, "HeadTextColor"=→"HeaderTextColor":u32, "FrameColor"=→"FrameColor":u32, "FrameThickness"=→"FrameThickness(1)":i32, "Header"=w26:u8[][], "ShouldHaveHeader"=w15:bool, "HeaderBkColor"=→"HeaderBkColor":u32, "Body"=w7:u8[][], "BodyBkColor"=→"BodyBkColor":u32, "SplitterAtRow"=w30:i32, "HeadText(OCR)"=→"HeadText(OCR)":string, "BodyText(OCR)"=→"BodyText(OCR)":string, "Splitter0px"=→"Splitter0px":bool)
  "BodyIcon" <- w7
  n213 = In Range and Coerce(upper limit=25 ("x"), x=w30, lower limit=2) -> (In Range?=w24:bool)  [unwired: 1 out]
  "ValidHeaderIcon" <- w24
  n214 = Select(t=w7, s=w15, f=u8[][] []) -> (s? t:f=w13:u8[][])
  n215 = Index Array(array=w7, index (row)=13) -> (element=w5:u8[])  [unwired: 1 in]
  n216 = Select(t=w26, s=w24, f=w13) -> (s? t:f=→"HeaderIcon":u8[][])
  n217 = Equal?(x=w5, y=u8[] [0, 0, 255, 44, 44, 44, 44, 44, 44, 44, 44, 44, 44, 44, 44, 44, 44, 44, 131, 5, 131, 131, 0, 0, 0, 0, 0, 0, 0, 0] ("subarray")) -> (x = y?=w11:bool)
  n218 = Equal?(x=w5, y=u8[] [0, 0, 0, 0, 0, 86, 252, 153, 74, 117, 116, 117, 172, 43, 0, 0, 0, 0, 0, 0, 0, 0, 0, 0, 0, 0, 0, 0, 0, 0] ("subarray 2")) -> (x = y?=w8:bool)
  n219 = Equal?(x=w5, y=u8[] [0, 0, 0, 246, 199, 199, 206, 199, 200, 202, 230, 203, 200, 199, 199, 206, 165, 165, 165, 43, 0, 0, 0, 0, 0, 0, 0, 0, 0, 0] ("subarray")) -> (x = y?=w3:bool)
  n220 = Compound Arithmetic op=OR(w11, w8, w3) -> (→"DefaultIcon":bool)
